vi "Timing Report.vi"   [LabVIEW 2014]
uses:
  <vilib>/Utility/error.llb/DialogType.ctl
  <vilib>/Wiresmith Technology/LabVIEW CLI/CLI Class/CLI.lvclass
types:
  T1 = cluster{"build_number":i32, "build_times":dbl[], "test_name":string}
  T2 = cluster{"mean":dbl, "standard deviation":dbl, "calculated percentiles":dbl[], "slope":dbl, "max":dbl}
  T3 = typedef "DialogType.ctl" = u16
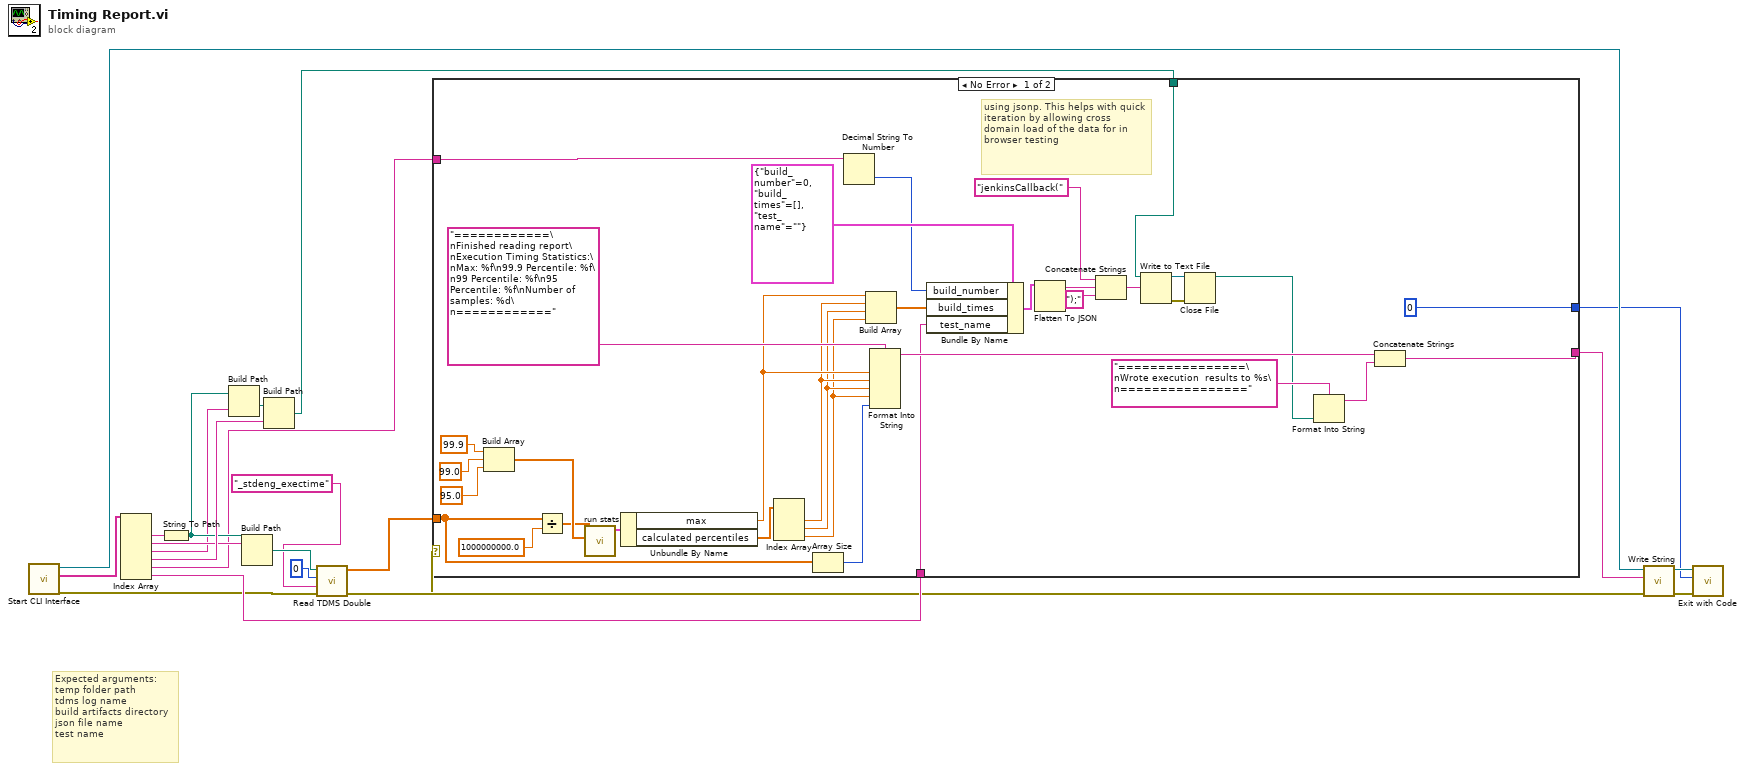
[diagram p0: block diagram]
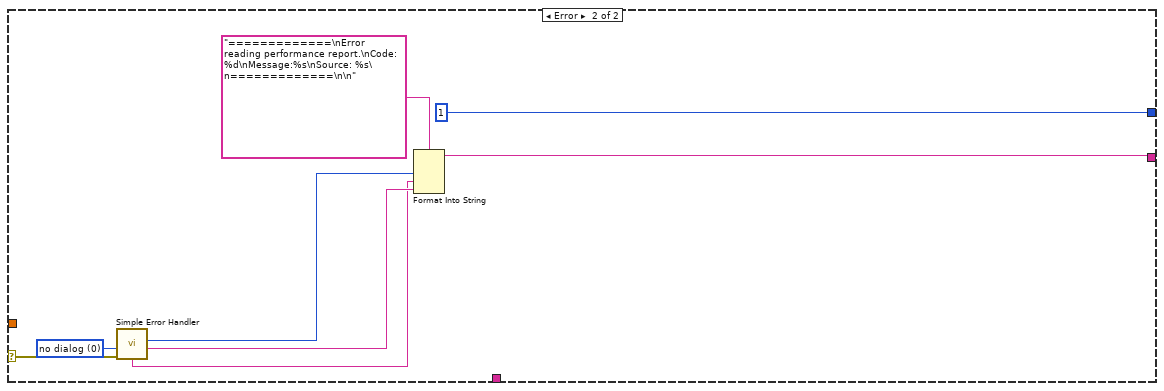
[diagram p2: hidden frame]
diagram:
  # "Expected arguments:\ntemp folder path\ntdms log name\nbuild artifacts directory\njson file name\ntest name"
  n1 = call <vilib>:"Start CLI Interface.vi"() -> ("error out"=w5:errorcluster, "Custom Parameters"=w21:string[], "CLI out"=w16:refnum<class "CLI.lvclass">)  [unwired: 9 in]
  n2 = Index Array(array=w21) -> (element #1=w20:string, element #2=w10:string, element #3=w9:string, element #4=w14:string, element #5=w8:string, element #6=w7:string)  [unwired: 6 in]
  n3 = String To Path(string=w20) -> (path=w11:path)
  n4 = Build Path(base path=w11, name or relative path=w9) -> (appended path=w12:path)
  n5 = Build Path(base path=w11, name or relative path=w10) -> (appended path=w6:path)
  n6 = Build Path(base path=w12, name or relative path=w14) -> (appended path=w13:path)
  n7 = call "Read TDMS Double.vi"("error in (no error)"=w5, "channel name(s) in"="_stdeng_exectime", "offset (0)"=i64 0, "file path"=w6) -> ("error out"=w2:errorcluster, "Data"=w1:dbl[])  [unwired: 6 in]
  n8 = case shown="No Error" w2 {
    selector: w2 -> [_ w60]
    tunnel: w1 -> [w22 _]
    tunnel: [w51 w56] -> w17
    tunnel: [0 ("Exit Code (0)") 1 ("Exit Code (0)")] -> w15
    tunnel: w13 -> [w48 _]
    tunnel: w8 -> [w40 _]
    tunnel: w7 -> [w34 _]
    frame No Error {
      # "using jsonp. This helps with quick iteration by allowing cross domain load of the data for in browser testing"
      n9 = Build Array(99.9 ("p"), 99.0 ("p"), 95.0 ("p")) -> (w33:dbl[])
      n10 = Divide(x=w22, y=1000000000.0) -> (x/y=w23:dbl[])
      n11 = call "run stats.vi"("percentiles"=w33, "Data"=w23) -> ("stats out"=w29:T2)  [unwired: 9 in]
      n12 = Unbundle By Name(w29) -> ("max"=w28:dbl, "calculated percentiles"=w27:dbl[])
      n13 = Index Array(array=w27) -> (element #1=w26:dbl, element #2=w25:dbl, element #3=w24:dbl)  [unwired: 3 in]
      n14 = Array Size(array=w22) -> (size(s)=w35:i32)
      n15 = Decimal String To Number(string=w40) -> (number=w38:i32)  [unwired: 2 in, 1 out]
      n16 = Build Array(w28, w26, w25, w24) -> (w37:dbl[])
      n17 = Format Into String(format string="============\nFinished reading report\nExecution Timing Statistics:\nMax: %f\n99.9 Percentile: %f\n99 Percentile: %f\n95 Percentile: %f\nNumber of samples: %d\n============", w28, w26, w25, w24, w35) -> (resulting string=w50:string)  [unwired: 2 in, 1 out]
      n18 = Bundle By Name(cluster=T1 {"build_number"=0, "build_times"=[], "test_name"=""}, "build_number"=w38, "build_times"=w37, "test_name"=w34) -> (w36:T1)
      n19 = Flatten To JSON(anything=w36) -> (JSON string=w43:string)  [unwired: 2 in, 1 out]
      n20 = Concatenate Strings("jenkinsCallback(" ("string"), w43, ");" ("string")) -> (w44:string)
      n21 = Write to Text File(file (use dialog)=w48, text=w44) -> (refnum out=w46:refnum<file>, error out=w47:errorcluster)  [unwired: 2 in, 1 out]
      n22 = Close File(refnum=w46, error in=w47) -> (path=w45:path)  [unwired: 1 out]
      n23 = Format Into String(format string="================\nWrote execution  results to %s\n================", w45) -> (resulting string=w49:string)  [unwired: 2 in, 1 out]
      n24 = Concatenate Strings(w50, w49) -> (w51:string)
    }
    frame Error {
      w61 = T3 0 items=["no dialog", "OK message", "continue or stop message", "OK message + warnings", "continue/stop + warnings"] ("type of dialog (OK msg:1)")
      n25 = call <vilib>:"Simple Error Handler.vi"("type of dialog (OK msg:1)"=w61, "error in (no error)"=w60) -> ("code out"=w59:i32, "source out"=w58:string, "message"=w57:string)  [unwired: 3 in, 2 out]
      n26 = Format Into String(format string="=============\nError reading performance report.\nCode: %d\nMessage:%s\nSource: %s\n=============\n\n", w59, w57, w58) -> (resulting string=w56:string)  [unwired: 2 in, 1 out]
    }
  }
  n27 = call <vilib>:"Write String.vi"("error in (no error)"=w5, "Text to Write"=w17, "CLI in"=w16) -> ("error out"=w19:errorcluster, "CLI out"=w18:refnum<class "CLI.lvclass">)  [unwired: 7 in]
  n28 = call <vilib>:"Exit with Code.vi"("error in (no error)"=w19, "Exit Code (0)"=w15, "CLI in"=w18) -> ()  [unwired: 8 in, 1 out]
